vi "Update Method Accessor.vi"(6 "accessor type":T1="Get", 7 "library":refnum<vi>, 8 "error in (no error)":errorcluster, 9 "method message metadata name":string, 10 "rpc method name":string, 11 "server class in":refnum<vi>) -> (0 "error out":errorcluster, 3 "server class out":refnum<vi>)   [LabVIEW 2019, in "gRPC Template Creation Utility.lvlib"]
uses:
  gRPC Template Creation Utility.lvlib
  TypeDefs/Method Accessor Type.ctl
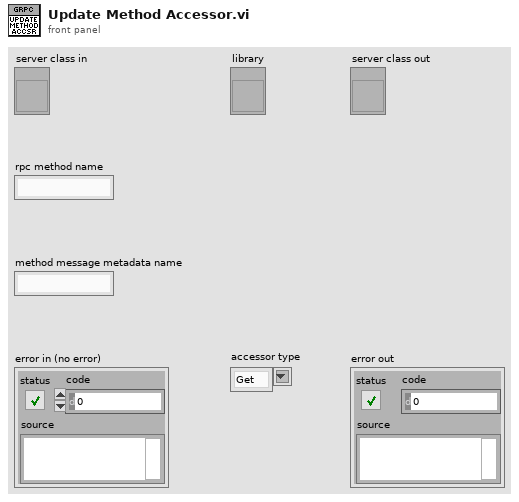
[diagram p1: front panel]
types:
  T1 = typedef "gRPC Template Creation Utility.lvlib/Method Accessor Type.ctl" = string
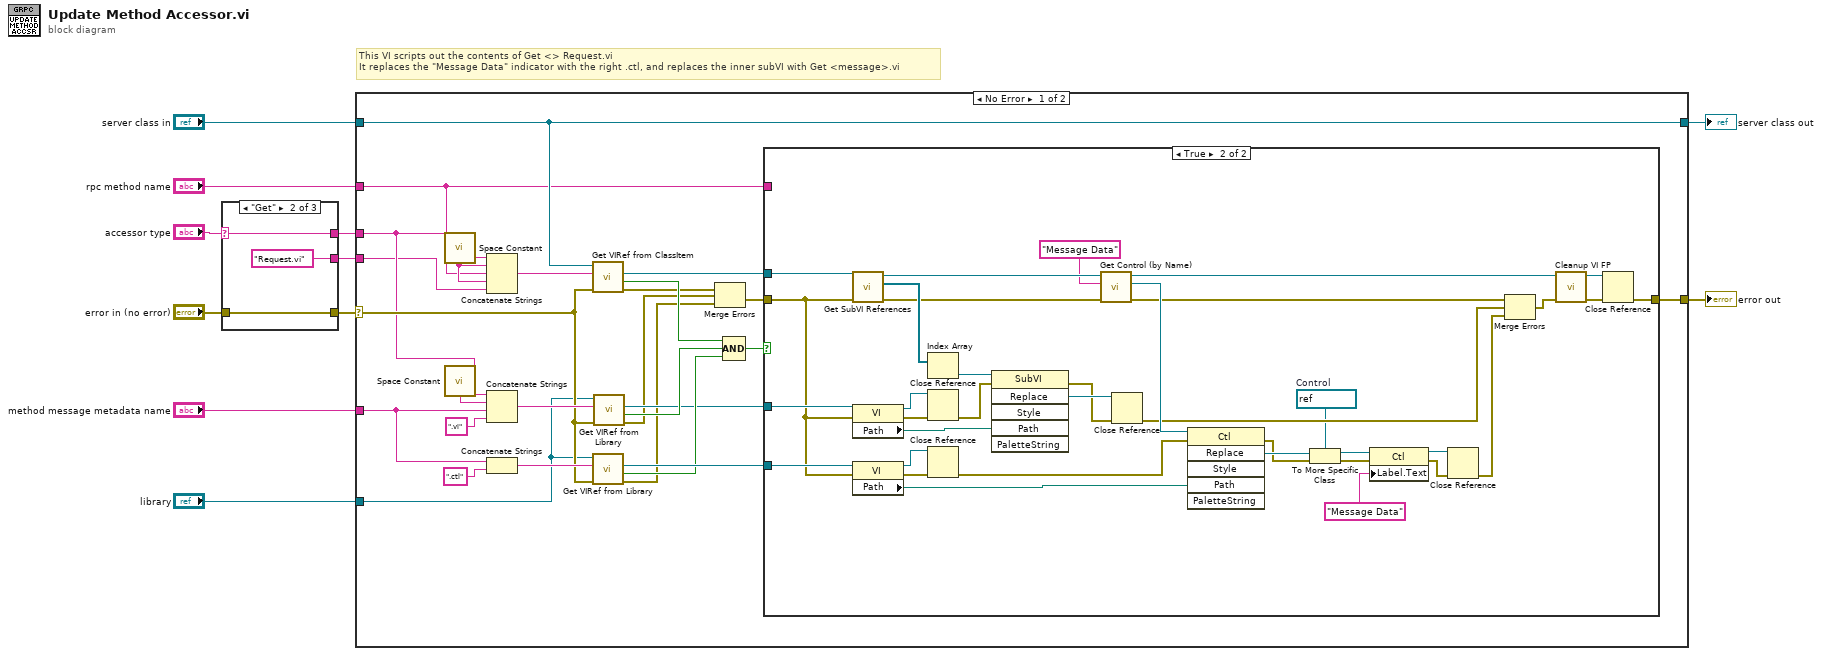
[diagram p0: block diagram]
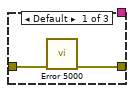
[diagram p2: hidden frame]
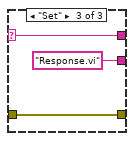
[diagram p3: hidden frame]
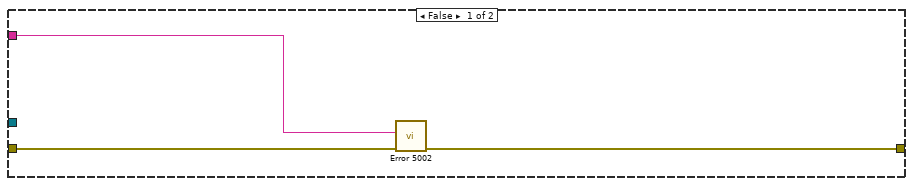
[diagram p4: hidden frame]
diagram:
  # "This VI scripts out the contents of Get <> Request.vi\nIt replaces the \"Message Data\" indicator with the right .ctl, and replaces the inner subVI with Get <message>.vi"
  n1 = case shown="\"Get\"" "accessor type" {
    selector: "accessor type" -> [_ w16 w19]
    tunnel: [_ w16 w19] -> w2
    tunnel: [_ "Request.vi" ("string") "Response.vi" ("string")] -> w1
    tunnel: "error in (no error)" -> [w13 w14 w17]
    tunnel: [w12 w14 w17] -> w3
    frame Default {
      n2 = call "Error 5000.vi"("error in (no error)"=w13) -> ("error out"=w12:errorcluster)  [unwired: 10 in]
    }
    frame "Get" {
    }
    frame "Set" {
    }
  }
  n3 = case shown="No Error" w3 {
    selector: w3 -> [w30 w86]
    tunnel: "server class in" -> [w24 w85]
    tunnel: "method message metadata name" -> [w38 _]
    tunnel: "rpc method name" -> [w23 _]
    tunnel: [w25 w86] -> w8
    tunnel: [w24 w85] -> w7
    tunnel: "library" -> [w22 _]
    tunnel: w2 -> [w21 _]
    tunnel: w1 -> [w20 _]
    frame No Error {
      n4 = call <vilib>:"Space Constant.vi"() -> ("String"=w31:string)
      n5 = call <vilib>:"Space Constant.vi"() -> ("String"=w32:string)
      n6 = Concatenate Strings(w21, w31, w23, w31, w20) -> (w35:string)
      n7 = Concatenate Strings(w21, w32, w38, ".vi" ("string")) -> (w34:string)
      n8 = Concatenate Strings(w38, ".ctl" ("string")) -> (w40:string)
      n9 = call "Get VIRef from ClassItem.vi"("error in (no error)"=w30, "Item Name"=w35, "LVClassLibrary in"=w24) -> ("error out"=w29:errorcluster, "Found ?"=w41:bool, "VIref out"=w36:refnum<vi>)  [unwired: 5 in, 1 out]
      n10 = call "Get VIRef from Library.vi"("error in (no error)"=w30, "Item Name"=w40, "Library"=w22) -> ("error out"=w26:errorcluster, "Found ?"=w43:bool, "VIref out"=w45:refnum<vi>)  [unwired: 5 in, 1 out]
      n11 = call "Get VIRef from Library.vi"("error in (no error)"=w30, "Item Name"=w34, "Library"=w22) -> ("error out"=w27:errorcluster, "Found ?"=w42:bool, "VIref out"=w37:refnum<vi>)  [unwired: 5 in, 1 out]
      n12 = Merge Errors(w29, w27, w26) -> (w28:errorcluster)
      n13 = Compound Arithmetic op=AND(w41, w42, w43) -> (w44:bool)
      n14 = case shown="True" w44 {
        tunnel: w36 -> [_ w82]
        tunnel: w37 -> [_ w81]
        tunnel: w45 -> [_ w77]
        tunnel: w28 -> [w48 w71]
        tunnel: [w47 w50] -> w25
        tunnel: w23 -> [w46 _]
        frame False {
          n15 = call "Error 5002.vi"("error in (no error)"=w48, "Method Name"=w46) -> ("error out"=w47:errorcluster)  [unwired: 9 in]
        }
        frame True {
          w60 = refnum<vi> refnum  # Control
          n16 = call "Get SubVI References.vi"("error in (no error)"=w71, "Owner vi in"=w82) -> ("error out"=w72:errorcluster, "SubVI refs"=w84:refnum<vi>[], "Owner vi out"=w75:refnum<vi>)  [unwired: 7 in]
          n17 = property class="VI"(reference=w81, error in=w71) -> (reference out=w67:refnum<vi>, error out=w68:errorcluster, "Path"=w80:path)
          n18 = property class="VI"(reference=w77, error in=w71) -> (reference out=w65:refnum<vi>, error out=w66:errorcluster, "Path"=w76:path)
          n19 = Index Array(array=w84) -> (element=w83:refnum<vi>)  [unwired: 1 in]
          n20 = Close Reference(reference=w67, error in (no error)=w68) -> (error out=w63:errorcluster)
          n21 = Close Reference(reference=w65, error in (no error)=w66) -> (error out=w64:errorcluster)
          n22 = invoke class="SubVI" method="Replace"(reference=w83, error in=w63, "Path"=w80) -> (error out=w78:errorcluster, "Replace"=w79:refnum<vi>)  [unwired: 3 in, 4 out]
          n23 = call "Get Control (by Name).vi"("error in (no error)"=w72, "Control Label"="Message Data" ("Constant Label"), "Owner VI in"=w75) -> ("error out"=w70:errorcluster, "Control Refnum"=w73:refnum<vi>, "Owner VI out"=w52:refnum<vi>)  [unwired: 5 in, 1 out]
          n24 = Close Reference(reference=w79, error in (no error)=w78) -> (error out=w69:errorcluster)
          n25 = invoke class="Ctl" method="Replace"(reference=w73, error in=w64, "Path"=w76) -> (error out=w61:errorcluster, "Replace"=w62:refnum<vi>)  [unwired: 3 in, 4 out]
          n26 = To More Specific Class(target class=w60, reference=w62, error in=w61) -> (specific class reference=w58:refnum<vi>, error out=w59:errorcluster)
          n27 = property class="Ctl"(reference=w58, error in=w59, "Label.Text"="Message Data") -> (reference out=w55:refnum<vi>, error out=w56:errorcluster)
          n28 = Close Reference(reference=w55, error in (no error)=w56) -> (error out=w54:errorcluster)
          n29 = Merge Errors(w70, w69, w54) -> (w53:errorcluster)
          n30 = call "Cleanup VI FP.vi"("error in"=w53, "vi in"=w52) -> ("error out"=w51:errorcluster, "vi out"=w49:refnum<vi>)  [unwired: 8 in]
          n31 = Close Reference(reference=w49, error in (no error)=w51) -> (error out=w50:errorcluster)
        }
      }
    }
    frame Error {
    }
  }
  "server class out" <- w7
  "error out" <- w8
